vi "Gen_TrajLib_Doc_TypeDef.vi"() -> ()   [LabVIEW 2019]
doc: "Generates and HTML file with the Description of every class, library, ctl, and vi in every open project. Creates separate documents for each library and virtual folder , and links to the top level document. In addition, for every VI shows connector pane. Saves the HTML file in folder <project folder>\\<project name> Documentation\\Documentation.html. erases previous content if any. \nDoes not create documentation for Documentation folder in project if exists. Does not create documentation for packed libraries in the project."
uses:
  Doc_Builder_SubVI/FileAndPath.ctl
  <vilib>/Utility/NIReport.llb/NI_report.lvclass
panel:
  out "Full Doc Path":path
  out "Full Input Path":path
  out "Finish Processed":bool
  in  "finish":bool
  out "ParamFoundBits":u32
  out "application name":string
  out "Cmd Line Read Error":errorcluster
  out "arguments":string[](array[string])
  out "Current Section":string
  out "File Index":i32
  out "File Count":i32
  in  "stop":bool
  out "Full Input File Name":path
  in  "GO":bool
  in  "Documentation Path":path=path "../HTML_Build_Work/Temp"
  in  "Library Path":path=path "../../FRC_LV_Trajectory_Library/TypeDef"
  # "DOCUMENT TYPE DEFINITIONS"
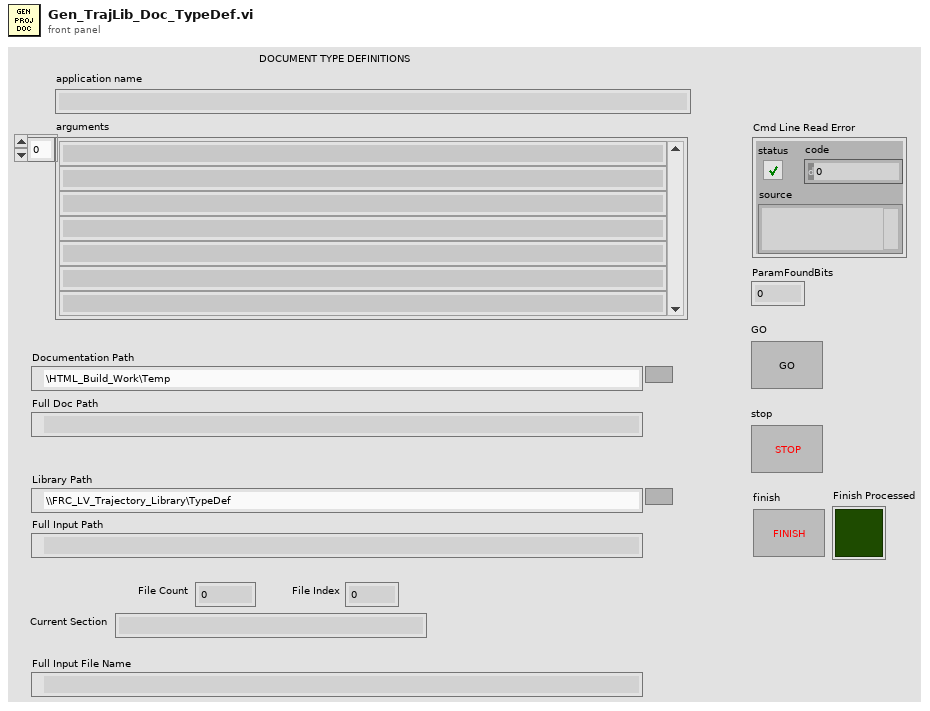
[diagram p1: front panel]
types:
  T1 = enum16{"Standard Report", "HTML", "Word", "Excel"}
  T2 = typedef "FileAndPath.ctl" = cluster{"FileName":string, "Library Path":path}
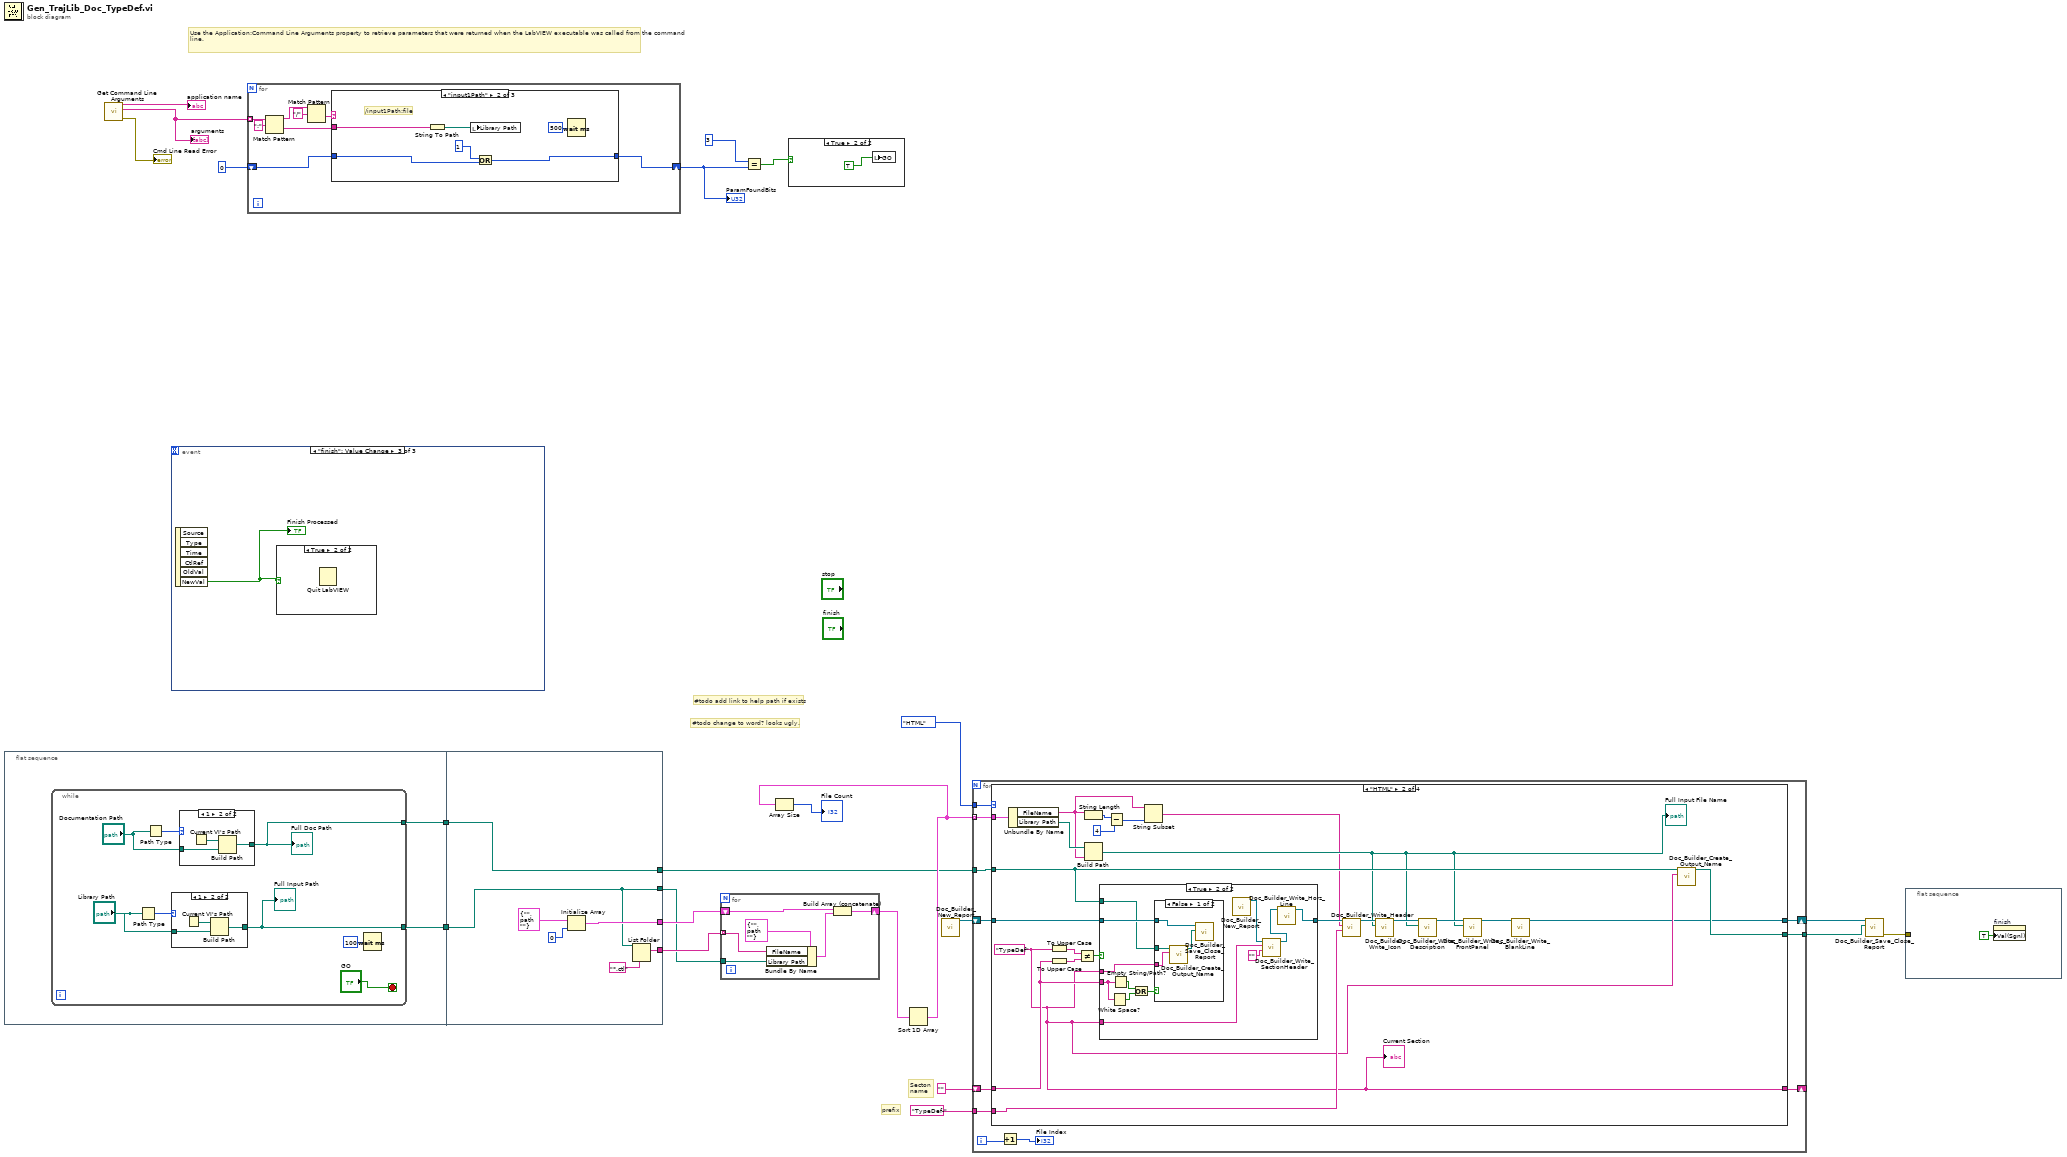
[diagram p0: block diagram]
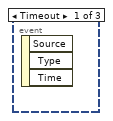
[diagram p4: hidden frame]
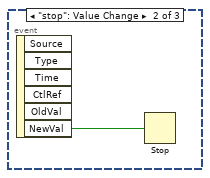
[diagram p5: hidden frame]
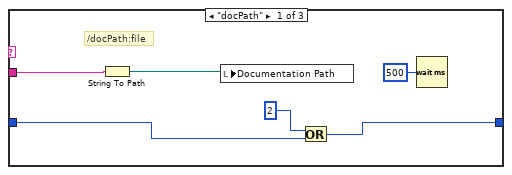
[diagram p8: hidden frame]
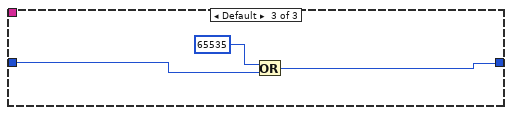
[diagram p9: hidden frame]
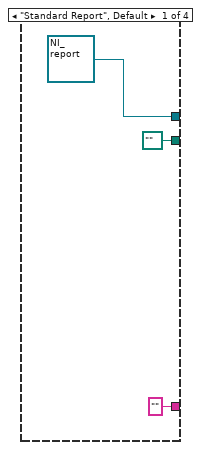
[diagram p10: hidden frame]
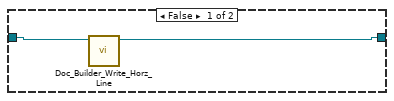
[diagram p11: hidden frame]
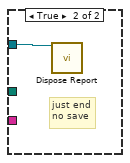
[diagram p12: hidden frame]
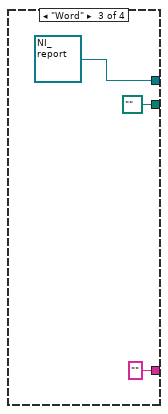
[diagram p13: hidden frame]
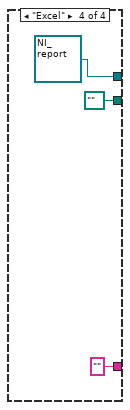
[diagram p14: hidden frame]
diagram:
  # "Use the Application:Command Line Arguments property to retrieve parameters that were returned when the LabVIEW executable was called from the command line."
  # "Secton \nname"
  # "prefix"
  # "#todo change to word? looks ugly."
  # "#todo add link to help path if exists"
  n1 = flat-sequence {
    tunnel: [w25] -> w2
    tunnel: [w24] -> w1
    tunnel: [w47] -> w20
    tunnel: [w45] -> w19
    tunnel: [w43] -> w4
    tunnel: [w42] -> w3
    tunnel: w2 -> [w43]
    tunnel: w1 -> [w42]
    frame #0 {
      n2 = while {
        tunnel: [w29] -> w25
        tunnel: [w26] -> w24
        stop <- "GO" stop-if-true
        n3 = Path Type(1:"Library Path") -> (0:w28:i16)
        n4 = Path Type(1:"Documentation Path") -> (0:w31:i16)
        n5 = case shown="1" w28 {
          tunnel: [w34 w36] -> w26
          tunnel: "Library Path" -> [w34 w35]
          frame 0, Default {
          }
          frame 1 {
            n6 = Current VI's Path() -> (path=w37:path)
            n7 = Build Path(base path=w37, name or relative path=w35) -> (appended path=w36:path)
          }
        }
        "Full Input Path" <- w26
        n8 = case shown="1" w31 {
          tunnel: [w38 w40] -> w29
          tunnel: "Documentation Path" -> [w38 w39]
          frame 0, Default {
          }
          frame 1 {
            n9 = Current VI's Path() -> (path=w41:path)
            n10 = Build Path(base path=w41, name or relative path=w39) -> (appended path=w40:path)
          }
        }
        "Full Doc Path" <- w29
        n11 = Wait (ms)(milliseconds to wait=u32 100) -> ()  [unwired: 1 out]
      }
    }
    frame #1 {
      n12 = Initialize Array(T2 {"FileName"="", "Library Path"=path ""} ("FileAndPath"), 0 ("dimension size")) -> (w45:T2[])
      n13 = List Folder(path=w42, pattern="*.ctl") -> (filenames=w47:string[])  [unwired: 2 in, 3 out]
    }
  }
  n14 = call <vilib>:"Get Command Line Arguments.vi"() -> ("error out"=→"Cmd Line Read Error":errorcluster, "arguments"=w9:string[], "application name"=→"application name":string)  [unwired: 9 in]
  "arguments" <- w9
  n15 = event shown="[2] \"finish\": Value Change" {
    selector: _ -> [_ _ _]
    dyn-events: _ -> [_ _ _]
    timeout: _ -> [_ _ _]
    event Timeout {
      n16 = event-data() -> ()  [unwired: 1 in, 3 out]
    }
    event "stop": Value Change {
      n17 = event-data() -> ("NewVal"=w49:bool)  [unwired: 1 in, 5 out]
      n18 = Stop(stop? (T)=w49) -> ()
    }
    event "finish": Value Change {
      n19 = event-data() -> ("NewVal"=w50:bool)  [unwired: 1 in, 5 out]
      "Finish Processed" <- w50
      n20 = case shown="True" w50 {
        frame False {
        }
        frame True {
          n21 = Quit LabVIEW() -> ()  [unwired: 1 in]
        }
      }
    }
  }
  n22 = for {
    tunnel: w9 -> [w57] mode=indexing
    shift-right: [w51] -> w8
    shift-left: u32 0 -> [w52]
    n23 = Match Pattern(string=w57, regular expression=":") -> (before substring=w55:string, after substring=w56:string)  [unwired: 3 out]
    n24 = Match Pattern(string=w55, regular expression="/") -> (after substring=w53:string)  [unwired: 4 out]
    n25 = case shown="\"input1Path\"" w53 {
      tunnel: w56 -> [w64 w70 _]
      tunnel: [w61 w68 w71] -> w51
      tunnel: w52 -> [w62 w69 w72]
      frame "docPath" {
        # "/docPath:file"
        n26 = String To Path(string=w64) -> (path=w60:path)
        n27 = local write "Documentation Path"(w60) -> ()
        n28 = Or(x=u32 2, y=w62) -> (x .or. y?=w61:u32)
        n29 = Wait (ms)(milliseconds to wait=u32 500) -> ()  [unwired: 1 out]
      }
      frame "input1Path" {
        # "/input1Path:file"
        n30 = String To Path(string=w70) -> (path=w66:path)
        n31 = local write "Library Path"(w66) -> ()
        n32 = Or(x=u32 1, y=w69) -> (x .or. y?=w68:u32)
        n33 = Wait (ms)(milliseconds to wait=u32 500) -> ()  [unwired: 1 out]
      }
      frame Default {
        n34 = Or(x=u32 65535, y=w72) -> (x .or. y?=w71:u32)
      }
    }
  }
  "ParamFoundBits" <- w8
  n35 = for {
    tunnel: w20 -> [w79] mode=indexing
    tunnel: w3 -> [w78]
    shift-right: [w77] -> w13
    shift-left: w19 -> [w76]
    n36 = Bundle By Name(cluster=T2 {"FileName"="", "Library Path"=path ""} ("FileAndPath"), "FileName"=w79, "Library Path"=w78) -> (w74:T2)
    n37 = Build Array (concatenate)(w76, w74) -> (w77:T2[])
  }
  n38 = Equal?(x=u32 3, y=w8) -> (x = y?=w6:bool)
  n39 = case shown="True" w6 {
    frame False {
    }
    frame True {
      n40 = local write "GO"(TRUE ("GO")) -> ()
    }
  }
  n41 = Sort 1D Array(array=w13) -> (sorted array=w18:T2[])
  n42 = Array Size(array=w18) -> (size(s)=→"File Count":i32)
  n43 = call "Doc_Builder_New_Report.vi"() -> ("NI_report out"=w17:refnum<class "NI_report.lvclass">)  [unwired: 11 in]
  n44 = for {
    tunnel: w18 -> [w90] mode=indexing
    tunnel: T1."HTML" ("report type") -> [w91]
    tunnel: w4 -> [w89]
    tunnel: "TypeDef-" ("string") -> [w86]
    shift-right: [w82] -> w15
    shift-left: w17 -> [w85]
    shift-right: [w81] -> _
    shift-left: "" ("string") -> [w84]
    tunnel: [w83] -> w14
    i -> [w88]
    n45 = case shown="\"HTML\"" w91 {
      tunnel: w90 -> [_ w112 _ _]
      tunnel: w89 -> [_ w103 _ _]
      tunnel: w86 -> [_ w100 _ _]
      tunnel: w85 -> [_ w107 _ _]
      tunnel: w84 -> [_ w104 _ _]
      tunnel: [path "" ("Full Report Name") w105 path "" ("Full Report Name") path "" ("Full Report Name")] -> w83
      tunnel: [refnum<class "NI_report.lvclass"> refnum ("report out") w95 refnum<class "NI_report.lvclass"> refnum ("report out") refnum<class "NI_report.lvclass"> refnum ("report out")] -> w82
      tunnel: ["" ("FileName") w97 "" ("FileName") "" ("FileName")] -> w81
      frame "Standard Report", Default {
      }
      frame "HTML" {
        w97 = "TypeDef" ("string")
        n46 = Unbundle By Name(w112) -> ("FileName"=w110:string, "Library Path"=w111:path)
        n47 = To Upper Case(1:w97) -> (0:w109:string)
        n48 = To Upper Case(1:w104) -> (0:w108:string)
        n49 = Not Equal?(x=w109, y=w108) -> (x != y?=w98:bool)
        n50 = Build Path(base path=w111, name or relative path=w110) -> (appended path=w101:path)
        "Full Input File Name" <- w101
        n51 = String Length(string=w110) -> (length=w117:i32)
        n52 = case shown="True" w98 {
          tunnel: w107 -> [w119 w128]
          tunnel: [w118 w125] -> w106
          tunnel: w104 -> [_ w126]
          tunnel: w103 -> [_ w127]
          tunnel: w97 -> [_ w122]
          tunnel: w97 -> [_ w121]
          frame False {
            n53 = call "Doc_Builder_Write_Horz_Line.vi"("NI_report in"=w119) -> ("NI_report out"=w118:refnum<class "NI_report.lvclass">)  [unwired: 10 in]
          }
          frame True {
            n54 = White Space?(1:w126) -> (0:w130:bool)
            n55 = Empty String/Path?(string/path=w126) -> (empty?=w129:bool)
            n56 = Or(x=w129, y=w130) -> (x .or. y?=w131:bool)
            n57 = case shown="False" w131 {
              tunnel: w128 -> [w135 w136]
              tunnel: w127 -> [w134 _]
              tunnel: w121 -> [w133 _]
              frame False {
                n58 = call "Doc_Builder_Create_Output_Name.vi"("Section Name"=w133, "Path"=w134) -> ("Full Report Name"=w132:path)  [unwired: 9 in]
                n59 = call "Doc_Builder_Save_Close_Report.vi"("appended path"=w132, "NI_report in"=w135) -> ()  [unwired: 9 in, 1 out]
              }
              frame True {
                # "just end\nno save"
                n60 = call-dynamic "Dispose Report.vi"("report in"=w136) -> ()  [unwired: 14 in, 1 out]
              }
            }
            n61 = call "Doc_Builder_New_Report.vi"() -> ("NI_report out"=w124:refnum<class "NI_report.lvclass">)  [unwired: 11 in]
            n62 = call "Doc_Builder_Write_SectionHeader.vi"("Prefix String"="", "Section Name"=w122, "NI_report in"=w124) -> ("NI_report out"=w123:refnum<class "NI_report.lvclass">)  [unwired: 8 in]
            n63 = call "Doc_Builder_Write_Horz_Line.vi"("NI_report in"=w123) -> ("NI_report out"=w125:refnum<class "NI_report.lvclass">)  [unwired: 10 in]
          }
        }
        n64 = Subtract(x=w117, y=4) -> (x-y=w115:i32)
        n65 = String Subset(string=w110, length (rest)=w115) -> (substring=w99:string)  [unwired: 1 in]
        n66 = call "Doc_Builder_Write_Header.vi"("Prefix String"=w100, "Item Name"=w99, "NI_report in"=w106) -> ("NI_report out"=w114:refnum<class "NI_report.lvclass">)  [unwired: 8 in]
        n67 = call "Doc_Builder_Write_Icon.vi"("Input Item file path"=w101, "NI_report in"=w114) -> ("NI_report out"=w113:refnum<class "NI_report.lvclass">)  [unwired: 9 in]
        n68 = call "Doc_Builder_Write_Description.vi"("input item file path"=w101, "NI_report in"=w113) -> ("NI_report out"=w102:refnum<class "NI_report.lvclass">)  [unwired: 9 in]
        n69 = call "Doc_Builder_Write_FrontPanel.vi"("input item file path"=w101, "NI_report in"=w102) -> ("NI_report out"=w96:refnum<class "NI_report.lvclass">)  [unwired: 9 in]
        n70 = call "Doc_Builder_Write_BlankLine.vi"("NI_report in"=w96) -> ("NI_report out"=w95:refnum<class "NI_report.lvclass">)  [unwired: 10 in]
        n71 = call "Doc_Builder_Create_Output_Name.vi"("Section Name"=w97, "Path"=w103) -> ("Full Report Name"=w105:path)  [unwired: 9 in]
        "Current Section" <- w97
      }
      frame "Word" {
      }
      frame "Excel" {
      }
    }
    n72 = Increment(x=w88) -> (x+1=→"File Index":i32)
  }
  n73 = call "Doc_Builder_Save_Close_Report.vi"("appended path"=w14, "NI_report in"=w15) -> ("error out"=w5:errorcluster)  [unwired: 9 in]
  n74 = flat-sequence {
    tunnel: w5 -> [_]
    frame #0 {
      n75 = property on="finish" class="Bool (strict)"("Val(Sgnl)"=TRUE ("Value (Signaling)")) -> ()  [unwired: 2 in, 2 out]
    }
  }
